vi "Delete_Oldest.vi"(11 "Folder ready":path) -> ()   [LabVIEW 2025]
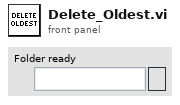
[diagram p1: front panel]
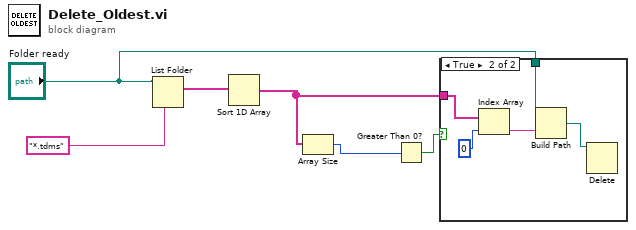
[diagram p0: block diagram]
diagram:
  n1 = List Folder(path="Folder ready", pattern="*.tdms") -> (filenames=w2:string[])  [unwired: 2 in, 3 out]
  n2 = Sort 1D Array(array=w2) -> (sorted array=w5:string[])
  n3 = Array Size(array=w5) -> (size(s)=w3:i32)
  n4 = Greater Than 0?(x=w3) -> (x > 0?=w4:bool)
  n5 = case shown="True" w4 {
    tunnel: w5 -> [_ w11]
    tunnel: "Folder ready" -> [_ w8]
    frame False {
    }
    frame True {
      n6 = Index Array(array=w11, index=0) -> (element=w9:string)
      n7 = Build Path(base path=w8, name or relative path=w9) -> (appended path=w7:path)
      n8 = Delete(path (use dialog)=w7) -> ()  [unwired: 4 in, 3 out]
    }
  }
